vi "icons-style-2.vi"() -> ()   [LabVIEW 2024]
panel:
  in  "String":string
  in  "Numeric":i32
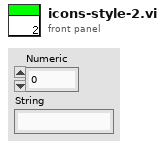
[diagram p1: front panel]
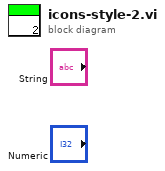
[diagram p0: block diagram]
diagram:
